vi "Add Connection Settings Channel.vi"(8 "error in (no error)":errorcluster, 11 "Modbus in":refnum<class "Modbus.lvclass">) -> (0 "error out":errorcluster, 3 "Modbus out":refnum<class "Modbus.lvclass">)   [LabVIEW 2026, in "Modbus.lvlib" / "Modbus.lvclass"]
uses:
  Modbus.lvclass
  <vilib>/FlexLogger/SDK/PluginSDK.lvlibp/PEFClasses/SDK/Channel/Data Type_v2.ctl
  <vilib>/FlexLogger/SDK/PluginSDK.lvlibp/PEFClasses/SDK/Producer Channel/Producer Channel.lvclass
  C:/Program Files/National Instruments/LabVIEW 2026/vi.lib/FlexLogger/SDK/PluginSDK.lvlibp/PEFClasses/SDK/Channel/Channel.lvclass
  Globals/Modbus Strings.vi
  <vilib>/FlexLogger/SDK/PluginSDK.lvlibp/PEFClasses/SDK/Producer Channel/Create Producer Channel_v2.vi
  <vilib>/FlexLogger/SDK/PluginSDK.lvlibp/PEFClasses/SDK/Channel/ParameterAccess/Write String.vi
  <vilib>/FlexLogger/SDK/PluginSDK.lvlibp/PEFClasses/SDK/Channel/ParameterAccess/Write I32.vi
  C:/Program Files/National Instruments/LabVIEW 2026/vi.lib/FlexLogger/SDK/PluginSDK.lvlibp/PEFClasses/SDK/Producer Channel/Producer Channel.lvclass
  C:/Program Files/National Instruments/LabVIEW 2026/vi.lib/FlexLogger/SDK/PluginSDK.lvlibp/PEFClasses/SDK/Plugin/Plugin.lvclass
  <vilib>/FlexLogger/SDK/PluginSDK.lvlibp
  <vilib>/FlexLogger/SDK/PluginSDK.lvlibp/PEFClasses/SDK/Channel/Channel.lvclass
  <vilib>/FlexLogger/SDK/PluginSDK.lvlibp/PEFClasses/SDK/Plugin/Plugin.lvclass
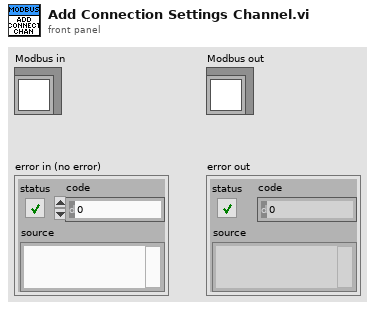
[diagram p1: front panel]
types:
  T1 = typedef "PluginSDK.lvlibp/Channel.lvclass/Data Type_v2.ctl" = u16
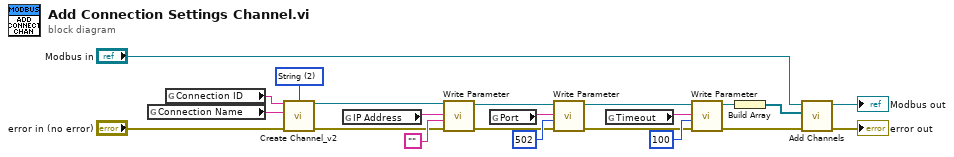
[diagram p0: block diagram]
diagram:
  w2 = T1 2 items=["Wfm (DBL)", "Wfm (Digital)", "String"] ("Data Type")
  n1 = global read "Modbus Strings.vi" "Connection Name"() -> (w20:string)
  n2 = global read "Modbus Strings.vi" "Connection ID"() -> (w19:string)
  n3 = call-poly <vilib>:"Create Channel_v2.vi"("Unique Channel Identifier"=w19, "Data Type"=w2, "Default Channel Name"=w20, "error in (no error)"="error in (no error)") -> ("Producer Channel"=w6:refnum<class "Producer Channel.lvclass">, "error out"=w7:errorcluster)  [unwired: 10 in]
  n4 = global read "Modbus Strings.vi" "IP Address"() -> (w8:string)
  n5 = call-poly <vilib>:"Write Parameter.vi"("error in (no error)"=w7, "Value"="", "Name"=w8, "Channel in"=w6) -> ("error out"=w11:errorcluster, "Channel out"=w10:refnum<class "Producer Channel.lvclass">)  [unwired: 6 in]
  n6 = global read "Modbus Strings.vi" "Port"() -> (w12:string)
  n7 = call-poly <vilib>:"Write Parameter.vi"("error in (no error)"=w11, "Value"=502, "Name"=w12, "Channel in"=w10) -> ("error out"=w15:errorcluster, "Channel out"=w14:refnum<class "Producer Channel.lvclass">)  [unwired: 6 in]
  n8 = global read "Modbus Strings.vi" "Timeout"() -> (w18:string)
  n9 = call-poly <vilib>:"Write Parameter.vi"("error in (no error)"=w15, "Value"=100 ("connect timeout ms"), "Name"=w18, "Channel in"=w14) -> ("error out"=w21:errorcluster, "Channel out"=w17:refnum<class "Producer Channel.lvclass">)  [unwired: 6 in]
  n10 = Build Array(w17) -> (w5:refnum<class "Producer Channel.lvclass">[])
  n11 = call <vilib>:"Add Channels.vi"("error in (no error)"=w21, "Channels"=w5, "Plugin in"="Modbus in") -> ("error out"=→"error out":errorcluster, "Plugin out"=→"Modbus out":refnum<class "Modbus.lvclass">)  [unwired: 7 in]
